vi "Close.vi"(8 "error in (no error)":errorcluster, 11 "ToastService in":refnum<class "ToastService.lvclass">) -> (0 "error out":errorcluster)   [LabVIEW 2026, in "ToastNotification.lvlib" / "ToastService.lvclass"]
doc: "Unregister the stored OnActivated callback, then close the service native reference. Cleanup runs independently of the incoming error and merges its errors with that error. Call once after the application stops accepting replies, outside the callback. Does not close a borrowed ToastBuilder or destroy caller-owned queues/events. There is no explicit in-flight callback drain or repeated-close guard in this phase. The example performs a final GC collection after all Close calls to release the observed .NET callback reservation."
uses:
  ToastService.lvclass
  ToastService.lvclass/ToastService.ctl
  Read event callback refnum.vi
  Read ActivationHandler.vi
  Read reference.vi
  C:/Users/loicw/Documents/LabVIEW/ToastNotifications/Sources/bins/Microsoft.Toolkit.Uwp.Notifications.dll
  bins/Microsoft.Toolkit.Uwp.Notifications.dll
  ActivationHandler/ActivationHandler.lvclass
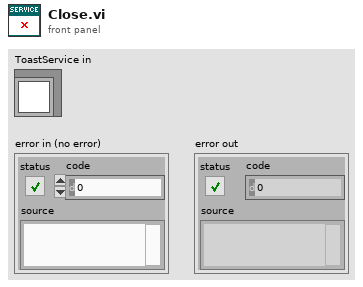
[diagram p1: front panel]
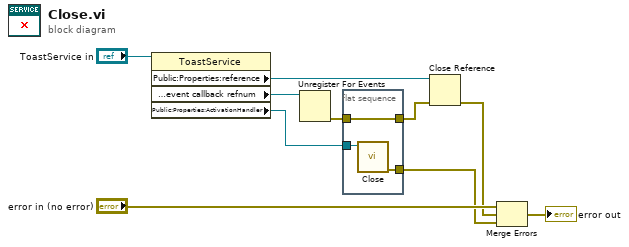
[diagram p0: block diagram]
diagram:
  n1 = property class="ToastService"(reference="ToastService in") -> ("Public:Properties:reference"=w7:refnum<k24>, "Private:Properties:event callback refnum"=w5:refnum<k27>, "Public:Properties:ActivationHandler"=w4:refnum<class "ActivationHandler.lvclass">)  [unwired: 1 in, 2 out]
  n2 = Unregister For Events(event registration refnum=w5) -> (error out=w1:errorcluster)  [unwired: 1 in]
  n3 = flat-sequence {
    tunnel: w4 -> [w13]
    tunnel: [w12] -> w3
    tunnel: [w11] -> w2
    tunnel: w1 -> [w11]
    frame #0 {
      n4 = call-dynamic "Close.vi"("ActivationHandler in"=w13) -> ("error out"=w12:errorcluster)  [unwired: 10 in]
    }
  }
  n5 = Close Reference(reference=w7, error in (no error)=w2) -> (error out=w6:errorcluster)
  n6 = Merge Errors("error in (no error)", w6, w3) -> (→"error out":errorcluster)
